vi "Start (Memory).vi"(7 "VolatusConfig":refnum<class "VolatusConfig.lvclass">, 8 "error in (no error)":errorcluster, 10 "Node Name":string) -> (0 "error out":errorcluster, 2 "MessageQ":refnum<class "MessageQ.lvclass">)   [LabVIEW 2020, in "Volatus.lvlib" / "Volatus Core.lvclass"]
uses:
  Volatus Core.lvclass
  Volatus Core.lvclass/Volatus Core.ctl
  Module/Module.lvclass
  VolatusAPI/VolatusAPI.lvclass
  VolatusConfig/VolatusConfig/VolatusConfig.lvclass
  Config Type.ctl
  VolatusConfig/Node/Node Config.lvclass
  MessageQ/MessageQ.lvclass
  C:/dev/lv20CE/relink/lv-volatus/Volatus/Module/Module.lvclass
  C:/dev/lv20CE/relink/lv-volatus/Volatus/Volatus Core/Volatus Core.lvclass
  C:/dev/lv20CE/relink/lv-volatus/VolatusConfig/VolatusConfigElement/VolatusConfigElement.lvclass
  C:/dev/lv20CE/relink/lv-volatus/VolatusConfig/Node/Node Config.lvclass
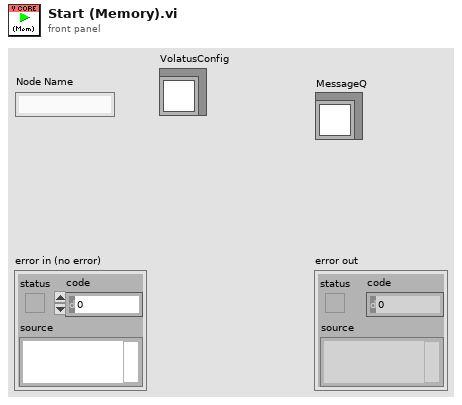
[diagram p1: front panel]
types:
  T1 = typedef "Volatus.lvlib/Volatus Core.lvclass/Config Type.ctl" = enum16{"App INI", "Memory", "Unconfigured"}
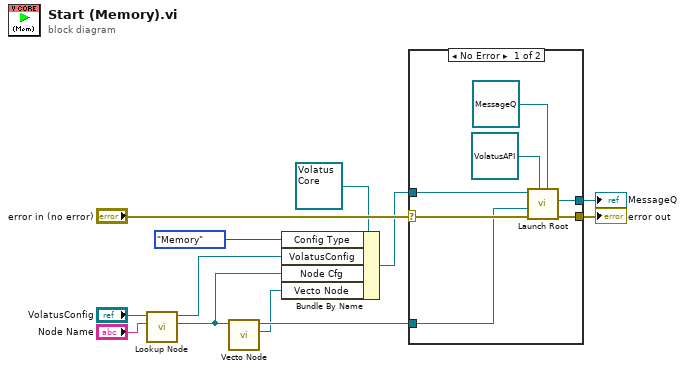
[diagram p0: block diagram]
diagram:
  n1 = call "Lookup Node.vi"("Node Name"="Node Name", "VolatusConfig in"="VolatusConfig") -> ("Node"=w3:refnum<class "Node Config.lvclass">, "VolatusConfig out"=w4:refnum<class "VolatusConfig.lvclass">)  [unwired: 7 in, 1 out]
  n2 = call "Vecto Node.vi"("Node in"=w3) -> ("Vecto Node"=w1:refnum<class "Node Config.lvclass">, "Node out"=w2:refnum<class "Node Config.lvclass">)  [unwired: 8 in, 1 out]
  n3 = Bundle By Name(cluster=refnum<class "Volatus Core.lvclass"> refnum ("Volatus Core in"), "Config Type"=Config_Type."Memory", "VolatusConfig"=w4, "Node Cfg"=w3, "Vecto Node"=w1) -> (w6:refnum<class "Volatus Core.lvclass">)
  n4 = case shown="No Error" "error in (no error)" {
    selector: "error in (no error)" -> [w19 w20]
    tunnel: [w18 w20] -> w11
    tunnel: [w17 _] -> w12
    tunnel: w6 -> [w16 _]
    tunnel: w2 -> [w14 _]
    frame No Error {
      n5 = call "Launch Root.vi"("Status Q"=refnum<class "MessageQ.lvclass"> refnum, "VolatusAPI"=refnum<class "VolatusAPI.lvclass"> refnum, "error in (no error)"=w19, "Config Element"=w14, "Module in"=w16) -> ("error out"=w18:errorcluster, "MessageQ"=w17:refnum<class "MessageQ.lvclass">)  [unwired: 5 in]
    }
    frame Error {
    }
  }
  "error out" <- w11
  "MessageQ" <- w12
